vi "Read Feed INI.vi"(8 "error in (no error)":errorcluster, 11 "feeds INI filepath":path) -> (0 "error out":errorcluster, 3 "feeds":T1[](array[typedef]))   [LabVIEW 2014]
doc: "Reads the feed data from the Feeds.ini file"
uses:
  Feed Info.ctl
  <vilib>/Utility/config.llb/Read Key (String).vi
  <vilib>/Utility/config.llb/NI_LVConfig.lvlib
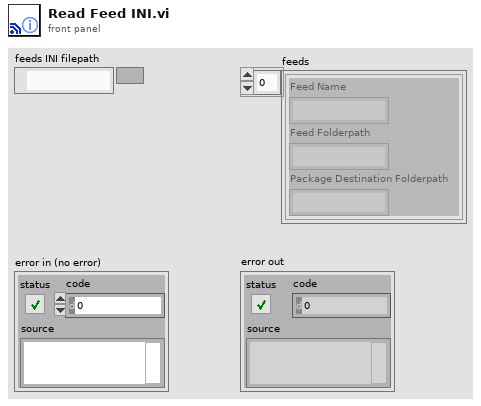
[diagram p1: front panel]
types:
  T1 = typedef "Feed Info.ctl" = cluster{"Feed Name":string, "Feed Folderpath":string, "Package Destination Folderpath":string}
  T2 = typedef "NI_LVConfig.lvlib/Config Data RefNum.ctl" = refnum<k1>
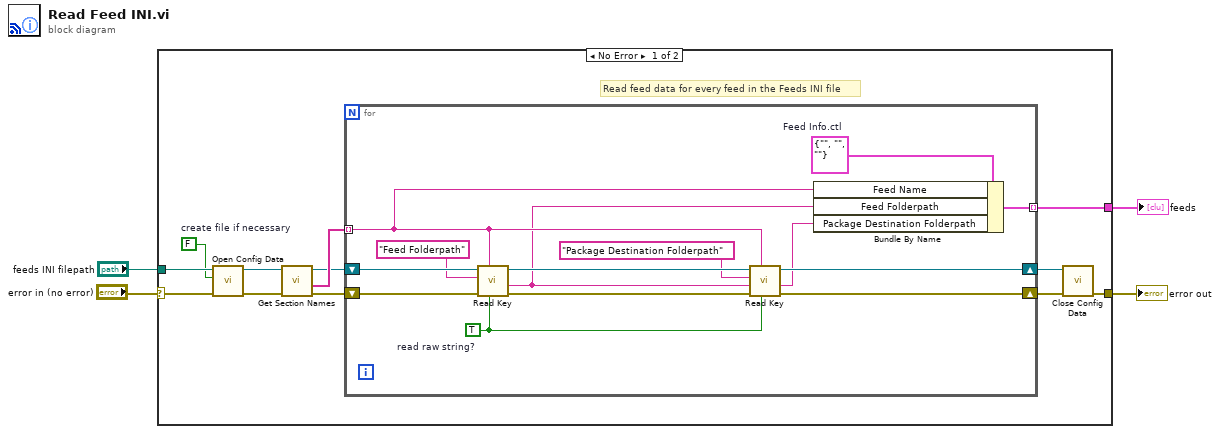
[diagram p0: block diagram]
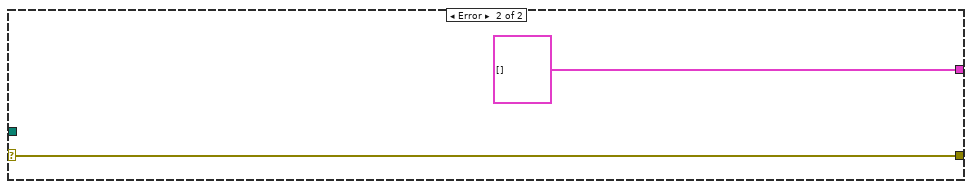
[diagram p2: hidden frame]
diagram:
  n1 = case shown="No Error" "error in (no error)" {
    selector: "error in (no error)" -> [w5 w32]
    tunnel: [w13 T1[] []] -> w4
    tunnel: "feeds INI filepath" -> [w10 _]
    tunnel: [w6 w32] -> w2
    frame No Error {
      w9 = FALSE  # create file if necessary
      # "Read feed data for every feed in the Feeds INI file"
      n2 = call <vilib>:"Open Config Data.vi"("error in (no error)"=w5, "create file if necessary (T)"=w9, "configuration file path"=w10) -> ("error out"=w8:errorcluster, "refnum"=w7:T2)  [unwired: 6 in, 1 out]
      n3 = call <vilib>:"Get Section Names.vi"("error in (no error)"=w8, "refnum"=w7) -> ("error out"=w14:errorcluster, "section names"=w12:string[], "refnum out"=w11:T2)  [unwired: 7 in]
      n4 = for {
        tunnel: w12 -> [w21] mode=indexing
        shift-right: [w22] -> w15
        shift-left: w11 -> [w30]
        tunnel: [w27] -> w13 mode=indexing
        shift-right: [w24] -> w16
        shift-left: w14 -> [w26]
        w17 = TRUE  # read raw string?
        w28 = T1 {"Feed Name"="", "Feed Folderpath"="", "Package Destination Folderpath"=""}  # Feed Info.ctl
        # "Read feed data for every feed in Feeds.ini"
        n5 = call-poly <vilib>:"Read Key.vi"("read raw string? (F)"=w17, "section"=w21, "error in (no error)"=w26, "key"="Feed Folderpath", "refnum"=w30) -> ("error out"=w25:errorcluster, "value"=w18:string, "refnum out"=w23:T2)  [unwired: 3 in, 1 out]
        n6 = call-poly <vilib>:"Read Key.vi"("read raw string? (F)"=w17, "section"=w21, "error in (no error)"=w25, "default value"=w18, "key"="Package Destination Folderpath", "refnum"=w23) -> ("error out"=w24:errorcluster, "value"=w19:string, "refnum out"=w22:T2)  [unwired: 2 in, 1 out]
        n7 = Bundle By Name(cluster=w28, "Feed Name"=w21, "Feed Folderpath"=w18, "Package Destination Folderpath"=w19) -> (w27:T1)
      }
      n8 = call <vilib>:"Close Config Data.vi"("error in (no error)"=w16, "refnum"=w15) -> ("error out"=w6:errorcluster)  [unwired: 8 in, 1 out]
    }
    frame Error {
    }
  }
  "feeds" <- w4
  "error out" <- w2
